vi "TEST - LVOOP Is Default Value.vi"(8 "error in (no error)":errorcluster) -> (0 "error out":errorcluster, 2 "Pass":bool)   [LabVIEW 2020, in "test_openg_array.lvlib"]
uses:
  LVOOP Data/Class 1/Class 1.lvclass
  test_openg_array.lvlib
  source/library/openg_variant.lvlib
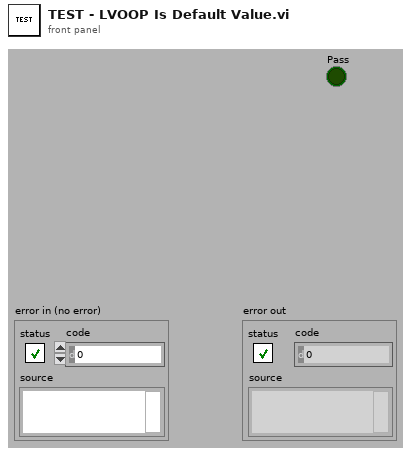
[diagram p1: front panel]
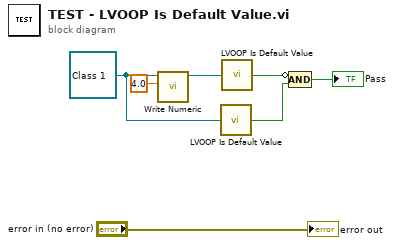
[diagram p0: block diagram]
diagram:
  w2 = refnum<class "Class 1.lvclass"> refnum ("Class 1.lvclass")
  n1 = call "Write Numeric.vi"("Numeric"=4.0, "Class 1 in"=w2) -> ("Class 1 out"=w3:refnum<class "Class 1.lvclass">)  [unwired: 9 in]
  n2 = call "LVOOP Is Default Value.vi"("Object"=w2) -> ("Is Default Value?"=w1:bool)
  n3 = call "LVOOP Is Default Value.vi"("Object"=w3) -> ("Is Default Value?"=w4:bool)
  n4 = Compound Arithmetic op=AND(invert w4, w1) -> (→"Pass":bool)
  "error out" <- "error in (no error)"
